vi "Copy template project to specified folder.vi"(11 "Test Case In":refnum<class "Runner Unit Test - Prepare Project.lvclass">) -> (0 "error out":errorcluster, 3 "Test Case Out":refnum<class "Runner Unit Test - Prepare Project.lvclass">)   [LabVIEW 2026, in "Runner Unit Test - Prepare Project.lvclass"]
uses:
  Runner Unit Test - Prepare Project.lvclass
  C:/Program Files/National Instruments/LabVIEW 2026/vi.lib/Astemes/LUnit/Test Case.lvclass
  Actors/Runner/Runner/Runner.lvclass
  Interfaces/IRunner/IRunner/Interfaces--cluster.ctl
  Interfaces/IProject Manager/IProject Manager.lvclass
  Interfaces/IFile Manager/IFile Manager.lvclass
  Interfaces/IPython Caller/IPython Caller.lvclass
  Interfaces/IElement Manager/IElement Manager.lvclass
  Interfaces/ILV File Creator/ILV File Creator.lvclass
  Interfaces/IHash Whitelist Handler/IHash Whitelist Handler.lvclass
  Actors/Mock Logger/Mock Logger/Mock Logger.lvclass
  C:/Program Files/National Instruments/LabVIEW 2026/vi.lib/ActorFramework/Actor/Actor.lvclass
  <vilib>/ActorFramework/Message Enqueuer/Message Enqueuer.lvclass/Message Enqueuer.ctl
  <vilib>/ActorFramework/Message Enqueuer/Enqueue.vi
  Mocks/Mock IFile Manager/Mock IFile Manager.lvclass
  C:/Program Files/National Instruments/LabVIEW 2026/vi.lib/Astemes/LMock/Mock.lvclass
  C:/Users/juanj/Documents/hasbun_wood_engineering/github/py2vi/labview/Interfaces/IFile Manager/IFile Manager.lvclass
  <vilib>/ActorFramework/Stop Msg/Stop Msg.lvclass
  C:/Program Files/National Instruments/LabVIEW 2026/vi.lib/ActorFramework/Message/Message.lvclass
  <vilib>/Astemes/LMock/One Identical Inputs.vi
  <vilib>/ActorFramework/Message Priority Queue/Priority Enqueue.vi
  Runner Unit Test - Prepare Project.lvclass/Runner Unit Test - Prepare Project.ctl
  C:/Users/juanj/Documents/hasbun_wood_engineering/github/py2vi/labview/Mocks/Mock IFile Manager/Mock IFile Manager.lvclass
  Interfaces/IRunner/IRunner/IRunner.lvclass
  <vilib>/ActorFramework/Actor/Actor.lvclass
  <vilib>/Astemes/LMock/LMock Verifier.lvclass
  <vilib>/Astemes/LMock/LMock.lvlib
  <vilib>/Astemes/LMock/LMock One.lvlib
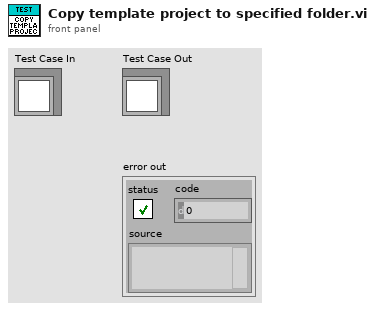
[diagram p1: front panel]
types:
  T1 = typedef "IRunner.lvlib/IRunner.lvclass/Interfaces--cluster.ctl" = cluster{"IProject Manager":refnum<class "IProject Manager.lvclass">, "IFile Manager":refnum<class "IFile Manager.lvclass">, "IPython Caller":refnum<class "IPython Caller.lvclass">, "IElement Manager":refnum<class "IElement Manager.lvclass">, "ILV File Creator":refnum<class "ILV File Creator.lvclass">, "IHash Whitelist Handler":refnum<class "IHash Whitelist Handler.lvclass">}
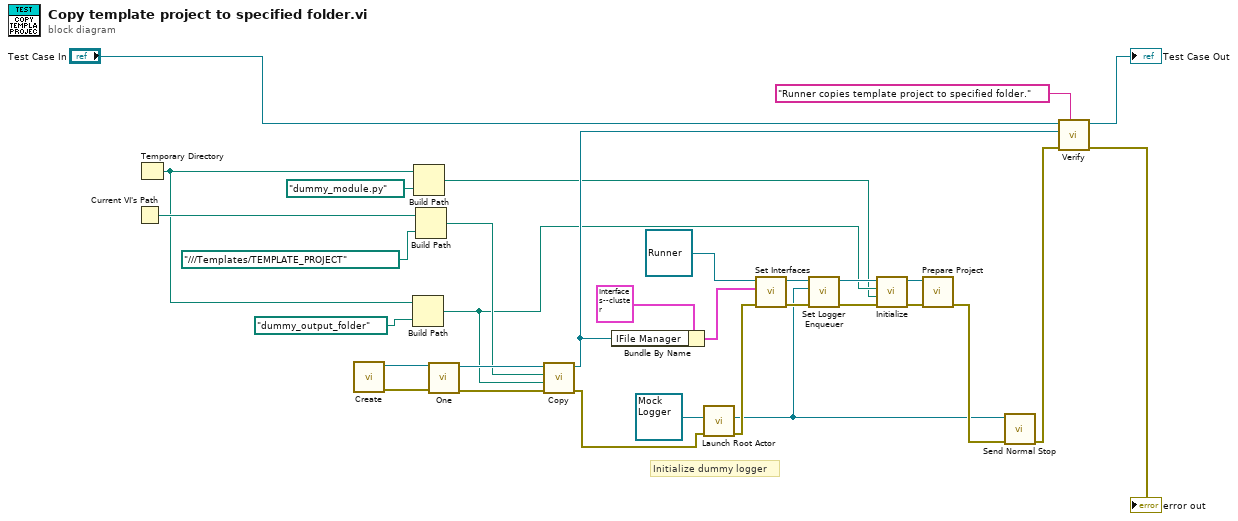
[diagram p0: block diagram]
diagram:
  # "Initialize dummy logger"
  n1 = Current VI's Path() -> (path=w7:path)
  n2 = Temporary Directory() -> (w1:path)
  n3 = call "Create.vi"() -> ("error out"=w31:errorcluster, "Mock Class Generator out"=w18:refnum<class "Mock IFile Manager.lvclass">)  [unwired: 10 in]
  n4 = Build Path(base path=w1, name or relative path=path "dummy_output_folder") -> (appended path=w5:path)
  n5 = Build Path(base path=w1, name or relative path=path "dummy_module.py") -> (appended path=w4:path)
  n6 = Build Path(base path=w7, name or relative path=path "../../../Templates/TEMPLATE_PROJECT") -> (appended path=w14:path)
  n7 = call-poly <vilib>:"One.vi"("error in (no error)"=w31, "Mock in"=w18) -> ("error out"=w30:errorcluster, "Mock out"=w17:refnum<class "Mock IFile Manager.lvclass">)  [unwired: 8 in]
  n8 = call-dynamic "Copy.vi"("error in"=w30, "Target Folder"=w5, "Source File"=w14, "IFile Manager in"=w17) -> ("error out"=w24:errorcluster, "IFile Manager out"=w15:refnum<class "Mock IFile Manager.lvclass">)  [unwired: 5 in, 1 out]
  n9 = Bundle By Name(cluster=T1 {"IProject Manager"=refnum, "IFile Manager"=refnum, "IPython Caller"=refnum, "IElement Manager"=refnum, "ILV File Creator"=refnum, "IHash Whitelist Handler"=refnum} ("Interfaces"), "IFile Manager"=w15) -> (w19:T1)
  n10 = call <vilib>:"Launch Root Actor.vi"("error in (no error)"=w24, "Actor"=refnum<class "Mock Logger.lvclass"> refnum ("Mock Logger.lvlib:Mock Logger.lvclass")) -> ("error out"=w29:errorcluster, "Actor's Enqueuer"=w12:refnum<class "Message Enqueuer.lvclass">)  [unwired: 8 in]
  n11 = call-dynamic "Set Interfaces.vi"("error in"=w29, "Interfaces"=w19, "Runner in"=refnum<class "Runner.lvclass"> refnum ("Runner.lvlib:Runner.lvclass")) -> ("error out"=w32:errorcluster, "Runner out"=w21:refnum<class "Runner.lvclass">)  [unwired: 7 in]
  n12 = call-dynamic "Set Logger Enqueuer.vi"("error in"=w32, "Logger"=w12, "Runner in"=w21) -> ("error out"=w26:errorcluster, "Runner out"=w9:refnum<class "Runner.lvclass">)  [unwired: 7 in]
  n13 = call-dynamic "Initialize.vi"("error in"=w26, "Python Module"=w4, "Output Folder"=w5, "G-CLI Runner in"=w9) -> ("error out"=w25:errorcluster, "G-CLI Runner out"=w8:refnum<class "Runner.lvclass">)  [unwired: 6 in]
  n14 = call-dynamic "Prepare Project.vi"("error in"=w25, "G-CLI Runner in"=w8) -> ("error out"=w28:errorcluster)  [unwired: 8 in, 1 out]
  n15 = call <vilib>:"Send Normal Stop.vi"("error in (no error)"=w28, "Message Enqueuer"=w12) -> ("error out"=w27:errorcluster)  [unwired: 9 in]
  n16 = call <vilib>:"Verify.vi"("Description"="Runner copies template project to specified folder.", "error in (no error)"=w27, "Mock"=w15, "LUnit Test Case In"="Test Case In") -> ("error out"=→"error out":errorcluster, "LUnit Test Case Out"=→"Test Case Out":refnum<class "Runner Unit Test - Prepare Project.lvclass">)  [unwired: 6 in]
